vi "update.cache.vi"(8 "error in":errorcluster, 11 "Run in":refnum<class "Run.lvclass">) -> (0 "error out":errorcluster, 3 "Run out":refnum<class "Run.lvclass">)   [LabVIEW 2020, in "Run.lvclass"]
uses:
  Run.lvclass
  Run.lvclass/Run.ctl
  Nominal Client/Nominal Client.lvclass/Nominal Client.ctl
  Nominal Client/create.authorization_header.vi
  Nominal Client/trace.payload_sent.vi
  Nominal Client/trace.payload_received.vi
  Nominal Client/error.vi
  Nominal Client/api_token.get.vi
  Nominal Client/trace.calling_method.vi
  <vilib>/JDP Science/JDP Science Common Utilities/Trim Whitespace__JDP.vi
  <vilib>/AdvancedString/1D String Array to Delimited String.vi
  Nominal Client/error.vi/859f8e04-e495-489b-b5b4-7ac163f56130.vi
  <vilib>/Utility/libraryn.llb/Get File Extension.vi
  Nominal Client/log_file.write.vi
  <vilib>/JDP Science/JSONtext/Get all Object Items.vi
  <vilib>/Utility/error.llb/Error Cluster From Error Code.vi
  <vilib>/JDP Science/JSONtext/JSON text to Variant.vi
  <vilib>/JDP Science/JSONtext/LVClass Serializer/JSONtext LVClass Serializer.lvclass
  <vilib>/addons/_JKI.lib/REST Client/classes/Response Headers/Response Headers.lvclass
  <vilib>/addons/_JKI.lib/REST Client/classes/REST Client/REST Client.lvclass
  Nominal Client/Nominal Client.lvclass
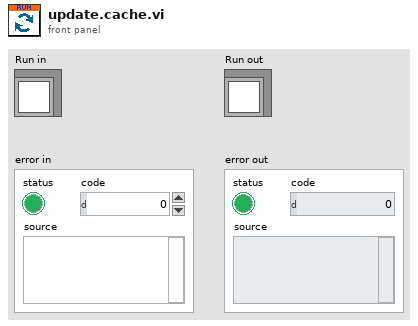
[diagram p1: front panel]
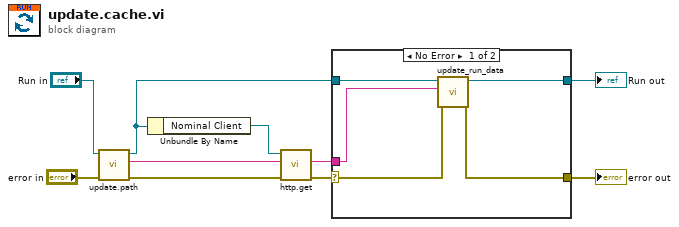
[diagram p0: block diagram]
diagram:
  n1 = call "update.path.vi"("error in"="error in", "Run"="Run in") -> ("error out"=w4:errorcluster, "path"=w8:string, "Run Out"=w10:refnum<class "Run.lvclass">)  [unwired: 7 in]
  n2 = Unbundle By Name(w10) -> ("Nominal Client"=w9:refnum<class "Nominal Client.lvclass">)
  n3 = call "http.get.vi"("error in"=w4, "Path"=w8, "Nominal Client in"=w9) -> ("error out"=w2:errorcluster, "Response"=w7:string)  [unwired: 5 in, 2 out]
  n4 = case shown="No Error" w2 {
    selector: w2 -> [w12 w17]
    tunnel: w10 -> [w15 w16]
    tunnel: w7 -> [w13 _]
    tunnel: [w14 w16] -> w6
    tunnel: [w11 w17] -> w1
    frame No Error {
      n5 = call "update_run_data.vi"("error in"=w12, "Run JSON"=w13, "Run in"=w15) -> ("error out"=w11:errorcluster, "Run out"=w14:refnum<class "Run.lvclass">)  [unwired: 7 in]
    }
    frame Error {
    }
  }
  "Run out" <- w6
  "error out" <- w1
